vi "test progress cancel by close.vi"(8 "error in (no error)":errorcluster) -> (0 "error out":errorcluster, 3 "body":string)   [LabVIEW 2020, in "MCP Server tests.lvlib"]
doc: "Cancellation by closing the stream (MCP 2026-07-28). A modern streamed tools/call of fake_tool_progress is sent over a raw TCP connection; as soon as the first notifications/progress event has arrived the client closes the connection. Report Progress.vi notices that the stream no longer drains and returns cancelled? TRUE, so the tool stops early: about 3 s later its record shows fewer than 10 steps and cancelled TRUE."
uses:
  MCP Server tests.lvlib
  b23f2e67-89a6-43fe-8e5c-3b8f47cb8976.vi
  <vilib>/JDP Science/JSONtext/Next JSON Value.vi
  <vilib>/JDP Science/JSONtext/String Subset.vi
  <vilib>/JDP Science/JSONtext/Parsing/Advance past next JSON Value (inlined COPY).vi
  <vilib>/JDP Science/JSONtext/Parsing/Advance past whitespace.vi
  <vilib>/JDP Science/JSONtext/Parsing/Advance past String.vi
  <vilib>/JDP Science/JSONtext/Parsing/Advance past Number.vi
  <vilib>/JDP Science/JSONtext/Parsing/Advance past Line Ending.vi
  <vilib>/JDP Science/JSONtext/Parsing/Parse Full Path or Item Name.vi
  <vilib>/JDP Science/JSONtext/Parsing/Advance past Array.vi
  <vilib>/JDP Science/JSONtext/Parsing/Advance past Object.vi
  <vilib>/JDP Science/JSONtext/support/Error Cluster From Code.vi
  <vilib>/JDP Science/JSONtext/Offset/Find Item Locations by Path.vi
  <vilib>/JDP Science/JSONtext/JSON text to Variant.vi
  <vilib>/JDP Science/JSONtext/LVClass Serializer/JSONtext LVClass Serializer.lvclass
  <vilib>/addons/_JKI Toolkits/Caraya/classes/Test/Test.lvclass
  <vilib>/addons/_JKI Toolkits/Caraya/classes/Assert/Assert.lvclass
  <vilib>/JDP Science/JSONtext/JSONtext.lvlib
panel:
  out "lookup error":errorcluster
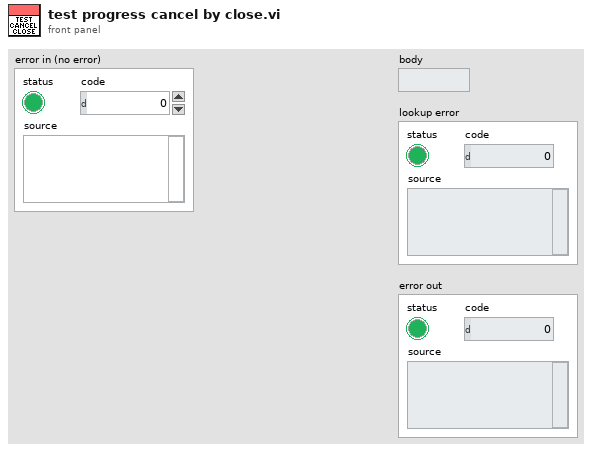
[diagram p1: front panel]
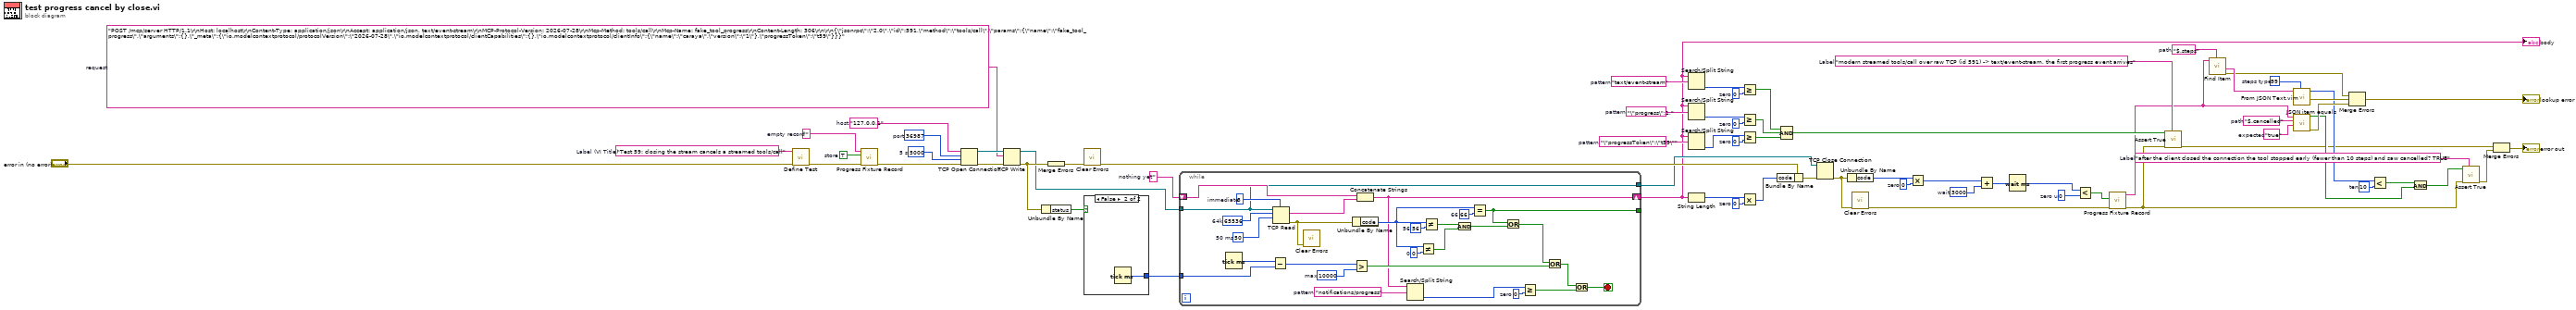
[diagram p0: block diagram]
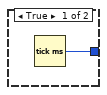
[diagram p2: hidden frame]
diagram:
  w6 = "after the client closed the connection the tool stopped early (fewer than 10 steps) and saw cancelled? TRUE"  # Label
  w22 = "modern streamed tools/call over raw TCP (id 591) -> text/event-stream, the first progress event arrives"  # Label
  w16 = "true"  # expected
  w17 = "$.cancelled"  # path
  w11 = 10  # ten
  w41 = 0  # zero
  w49 = "\"progressToken\":\"t59\""  # pattern
  w43 = 0  # zero
  w50 = "\"progress\":1,"  # pattern
  w45 = 0  # zero
  w51 = "text/event-stream"  # pattern
  w19 = 99  # steps type
  w21 = "$.steps"  # path
  w26 = u32 0  # zero u
  w29 = 3000  # wait
  w31 = 0  # zero
  w47 = 0  # zero
  w52 = ""  # nothing yet
  w59 = "POST /mcp/server HTTP/1.1\r\nHost: localhost\r\nContent-Type: application/json\r\nAccept: application/json, text/event-stream\r\nMCP-Protocol-Version: 2026-07-28\r\nMcp-Method: tools/call\r\nMcp-Name: fake_tool_progress\r\nContent-Length: 306\r\n\r\n{\"jsonrpc\":\"2.0\",\"id\":591,\"method\":\"tools/call\",\"params\":{\"name\":\"fake_tool_progress\",\"arguments\":{},\"_meta\":{\"io.modelcontextprotocol/protocolVersion\":\"2026-07-28\",\"io.modelcontextprotocol/clientCapabilities\":{},\"io.modelcontextprotocol/clientInfo\":{\"name\":\"caraya\",\"version\":\"1\"},\"progressToken\":\"t59\"}}}"  # request
  w62 = 5000  # 5 s
  w63 = u16 36987  # port
  w64 = "127.0.0.1"  # host
  w66 = TRUE  # store
  w67 = ""  # empty record
  w69 = "Test 59: closing the stream cancels a streamed tools/call"  # Label (VI Title)
  n1 = call <vilib>:"Define Test.vi"("error in (no error)"="error in (no error)", "Label (VI Title)"=w69) -> ("error out"=w65:errorcluster)  [unwired: 8 in, 1 out]
  n2 = call "Progress Fixture Record.vi"("error in"=w65, "set?"=w66, "record in"=w67) -> ("error out"=w61:errorcluster)  [unwired: 7 in, 1 out]
  n3 = TCP Open Connection(address=w64, remote port or service name=w63, timeout ms (60000)=w62, error in (no error)=w61) -> (connection ID=w60:refnum<k5>, error out=w58:errorcluster)  [unwired: 1 in]
  n4 = TCP Write(connection ID=w60, data in=w59, error in (no error)=w58) -> (connection ID out=w54:refnum<k5>, error out=w57:errorcluster)  [unwired: 1 in, 1 out]
  n5 = Unbundle By Name(w57) -> ("status"=w56:bool)
  n6 = Merge Errors(w57) -> (w55:errorcluster)
  n7 = call <vilib>:"Clear Errors.vi"("error in (no error)"=w55) -> ("error out"=w39:errorcluster)  [unwired: 5 in, 1 out]
  n8 = case shown="False" w56 {
    tunnel: [w70 w71] -> w53
    frame True {
      n9 = Tick Count (ms)() -> (millisecond timer value=w70:u32)
    }
    frame False {
      n10 = Tick Count (ms)() -> (millisecond timer value=w71:u32)
    }
  }
  n11 = while {
    tunnel: w54 -> [w73]
    tunnel: w53 -> [w95]
    shift-right: [w75] -> w3
    shift-left: w52 -> [w74]
    tunnel: [w73] -> w38
    tunnel: [w72] -> _
    stop <- w76 stop-if-true
    w82 = 0  # zero
    w86 = "notifications/progress"  # pattern
    w91 = u32 10000  # max
    w87 = 0  # 0
    w89 = 56  # 56
    w90 = 66  # 66
    w97 = u16 3  # immediate
    w98 = 50  # 50 ms
    w99 = 65536  # 64k
    n12 = Tick Count (ms)() -> (millisecond timer value=w96:u32)
    n13 = Subtract(x=w96, y=w95) -> (x-y=w92:u32)
    n14 = TCP Read(connection ID=w73, bytes to read=w99, 7:w97, 9:w98) -> (data out=w93:string, error out=w94:errorcluster)  [unwired: 1 in, 1 out]
    n15 = call <vilib>:"Clear Errors.vi"("error in (no error)"=w94) -> ()  [unwired: 5 in, 2 out]
    n16 = Unbundle By Name(w94) -> ("code"=w88:i32)
    n17 = Greater?(x=w92, y=w91) -> (0:w79:bool)
    n18 = Concatenate Strings(w74, w93) -> (w75:string)
    n19 = Search/Split String(string=w75, search string/char (-)=w86) -> (offset of match=w83:i32)  [unwired: 1 in, 2 out]
    n20 = Not Equal?(x=w88, y=w87) -> (x != y?=w84:bool)
    n21 = Not Equal?(x=w88, y=w89) -> (x != y?=w85:bool)
    n22 = And(x=w85, y=w84) -> (x .and. y?=w81:bool)
    n23 = Equal?(x=w88, y=w90) -> (x = y?=w72:bool)
    n24 = Or(x=w72, y=w81) -> (x .or. y?=w80:bool)
    n25 = Greater Or Equal?(x=w83, y=w82) -> (x >= y?=w77:bool)
    n26 = Or(x=w80, y=w79) -> (x .or. y?=w78:bool)
    n27 = Or(x=w78, y=w77) -> (x .or. y?=w76:bool)
  }
  "body" <- w3
  n28 = Search/Split String(string=w3, search string/char (-)=w51) -> (offset of match=w46:i32)  [unwired: 1 in, 2 out]
  n29 = Search/Split String(string=w3, search string/char (-)=w50) -> (offset of match=w44:i32)  [unwired: 1 in, 2 out]
  n30 = Search/Split String(string=w3, search string/char (-)=w49) -> (offset of match=w42:i32)  [unwired: 1 in, 2 out]
  n31 = String Length(string=w3) -> (length=w48:i32)
  n32 = Greater Or Equal?(x=w46, y=w45) -> (x >= y?=w36:bool)
  n33 = Greater Or Equal?(x=w44, y=w43) -> (x >= y?=w35:bool)
  n34 = Greater Or Equal?(x=w42, y=w41) -> (x >= y?=w34:bool)
  n35 = Multiply(x=w48, y=w47) -> (x*y=w40:i32)
  n36 = Bundle By Name(cluster=w39, "code"=w40) -> (w37:errorcluster)
  n37 = Compound Arithmetic op=AND(w36, w35, w34) -> (w23:bool)
  n38 = TCP Close Connection(connection ID=w38, error in (no error)=w37) -> (error out=w33:errorcluster)  [unwired: 1 in, 1 out]
  n39 = Unbundle By Name(w33) -> ("code"=w32:i32)
  n40 = call <vilib>:"Clear Errors.vi"("error in (no error)"=w33) -> ("error out"=w24:errorcluster)  [unwired: 5 in, 1 out]
  n41 = Multiply(x=w32, y=w31) -> (x*y=w30:i32)
  n42 = Add(x=w30, y=w29) -> (x+y=w28:i32)
  n43 = Wait (ms)(milliseconds to wait=w28) -> (millisecond timer value=w27:u32)
  n44 = Less?(x=w27, y=w26) -> (x < y?=w25:bool)
  n45 = call "Progress Fixture Record.vi"("error in"=w24, "set?"=w25) -> ("error out"=w7:errorcluster, "record out"=w18:string)  [unwired: 8 in]
  n46 = call <vilib>:"Assert True.vi"("Label"=w22, "error in (no error)"=w7, "True?"=w23) -> ("error out"=w5:errorcluster)  [unwired: 7 in, 1 out]
  n47 = call <vilib>:"Find Item.vi"("$Path or Item Name"=w21, "JSON"=w18) -> ("error out"=w15:errorcluster, "<JSON>"=w20:string)  [unwired: 6 in, 2 out]
  n48 = call "From JSON Text.vim"("Data Type and Default Value"=w19, "JSON"=w20) -> ("error out"=w14:errorcluster, "Data out"=w12:i32)  [unwired: 8 in]
  n49 = call "JSON item equals.vi"("expected"=w16, "path"=w17, "JSON"=w18) -> ("error out"=w13:errorcluster, "equal?"=w9:bool)  [unwired: 6 in, 1 out]
  n50 = Merge Errors(w15, w14, w13) -> (→"lookup error":errorcluster)
  n51 = Less?(x=w12, y=w11) -> (x < y?=w10:bool)
  n52 = And(x=w10, y=w9) -> (x .and. y?=w8:bool)
  n53 = call <vilib>:"Assert True.vi"("Label"=w6, "error in (no error)"=w7, "True?"=w8) -> ("error out"=w4:errorcluster)  [unwired: 7 in, 1 out]
  n54 = Merge Errors(w5, w4) -> (→"error out":errorcluster)
